vi "PauseResume.vi"(8 "error in":errorcluster, 10 "UI GUID":string, 11 "PauseResume Ref":refnum<vi>) -> (0 "error out":errorcluster, 3 "Data":string[][](array[string]))   [LabVIEW 2025, in "CAN-LIN Raw Bus Capture UI.lvlib"]
doc: "Get new data from the Table Buffer Queue, if the Plug-In is unpaused.\n\nDoes not wait for an element, only dequeues if elements are in the queue.\n\nIf the Update? is True then onyl checks the pause state. This means that if you want to ignore leftover packages when paused at shutdown, keep it on true."
uses:
  CAN-LIN Raw Bus Capture UI.lvlib
  Get Status.vi
  Dequeue Data.vi
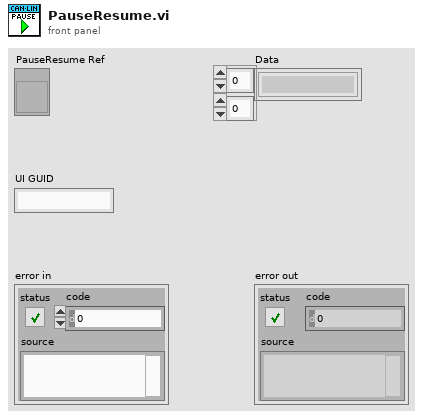
[diagram p1: front panel]
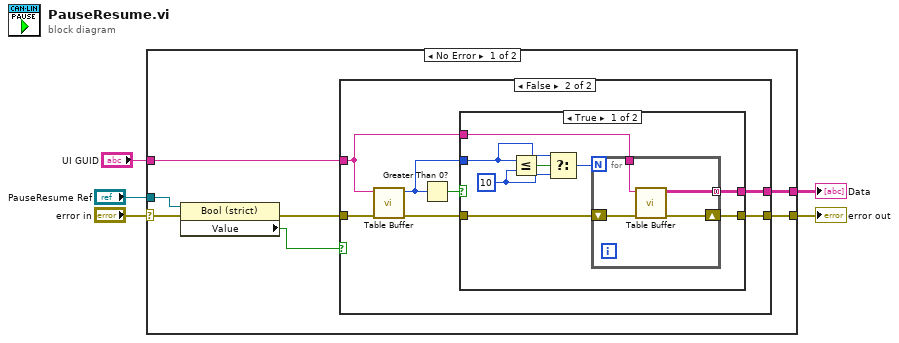
[diagram p0: block diagram]
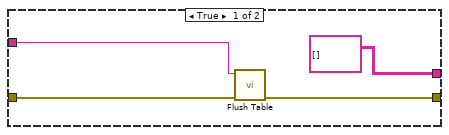
[diagram p2: hidden frame]
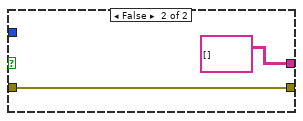
[diagram p3: hidden frame]
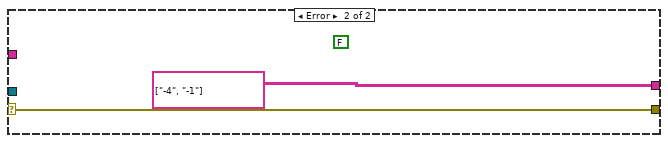
[diagram p4: hidden frame]
diagram:
  n1 = case shown="No Error" "error in" {
    selector: "error in" -> [w11 w39]
    tunnel: [w12 w39] -> w5
    tunnel: "PauseResume Ref" -> [w9 _]
    tunnel: [w8 string[][] [["-4", "-1"]] ("Data")] -> w2
    tunnel: "UI GUID" -> [w6 _]
    frame No Error {
      n2 = property class="Bool (strict)"(reference=w9, error in=w11) -> (error out=w10:errorcluster, "Value"=w7:bool)  [unwired: 1 out]
      n3 = case shown="False" w7 {
        tunnel: [w15 w23] -> w12
        tunnel: w10 -> [w14 w20]
        tunnel: [string[][] [] ("Data") w22] -> w8
        tunnel: w6 -> [w13 w17]
        frame True {
          n4 = call "Flush Table.vi"("error in"=w14, "UI GUID"=w13) -> ("error out"=w15:errorcluster)  [unwired: 9 in]
        }
        frame False {
          n5 = call-poly "Table Buffer.vi"("error in"=w20, "UI GUID"=w17) -> ("error out"=w21:errorcluster, "Messages"=w18:i32)  [unwired: 8 in]
          n6 = Greater Than 0?(x=w18) -> (x > 0?=w19:bool)
          n7 = case shown="True" w19 {
            tunnel: [w31 w36] -> w23
            tunnel: w21 -> [w30 w36]
            tunnel: [w25 string[][] [] ("Data")] -> w22
            tunnel: w18 -> [w27 _]
            tunnel: w17 -> [w24 _]
            frame True {
              w28 = 10 ("y")
              n8 = Less Or Equal?(x=w27, y=w28) -> (x <= y?=w29:bool)
              n9 = Select(t=w27, s=w29, f=w28) -> (s? t:f=w26:i32)
              n10 = for {
                N: w26 -> [_]
                shift-right: [w35] -> w31
                shift-left: w30 -> [w34]
                tunnel: [w33] -> w25 mode=concatenating
                tunnel: w24 -> [w32]
                n11 = call-poly "Table Buffer.vi"("error in"=w34, "UI GUID"=w32) -> ("error out"=w35:errorcluster, "Data"=w33:string[][])  [unwired: 8 in]
              }
            }
            frame False {
            }
          }
        }
      }
    }
    frame Error {
      (unwired) FALSE ("Value")
    }
  }
  "error out" <- w5
  "Data" <- w2
